vi "Open.vi"(4 "Help URL or File Path":string, 5 "Global Timeout [mSec] (-1)":i32=-1, 6 "Caller VI":refnum<vi>, 7 "Delay [mSec] (0)":u32, 8 "error in (no error)":errorcluster, 9 "Explorer Visible? (F)":bool, 10 "Window Title":string="Action Status", 11 "Bar in":refnum<class "Bar.lvclass">) -> (0 "error out":errorcluster, 3 "Bar out":refnum<class "Bar.lvclass">)   [LabVIEW 2015, in "Simple Progress Bar.lvlib" / "Bar.lvclass"]
doc: "Open the progress bar user interface.\n\n<b>Window Title</b> string will replace the title of the window.\n\n<b>Explorer Visible</b> if enabled will make Explorer button visible. The VI checks if the directory path exists when the event is thrown.\n\n<b>Caller VI</b> reference is used to display progression in the task bar icon (available from Microsoft Windows 7).\n\n<b>Delay</b> in mSec will delay window opening without delaying the process (asynchronous).\n\n<b>Global Timeout</b> duration in mSec will automatically close the window if the process has not finished before."
uses:
  Bar.lvclass
  Bar.lvclass/Bar.ctl
  Simple Progress Bar.lvlib
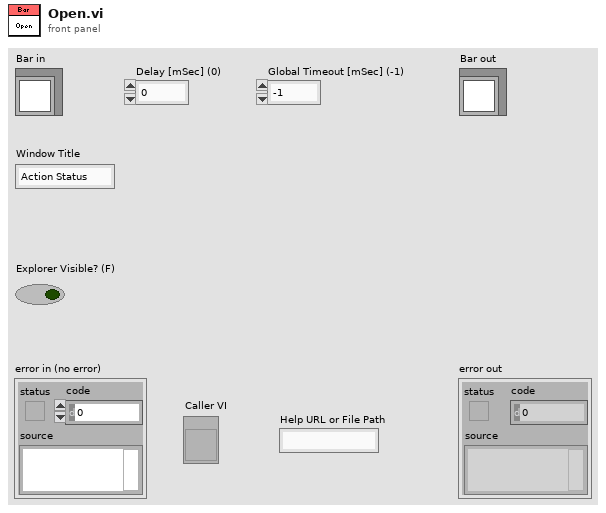
[diagram p1: front panel]
types:
  T1 = enum32{"Invalid", "Standard", "Closed", "Hidden", "Minimized", "Maximized"}
  T2 = typedef "Simple Progress Bar.lvlib/UI Events.ctl" = cluster{"Done":refnum<user-event>, "Cancel":refnum<user-event>, "Explore":refnum<user-event>}
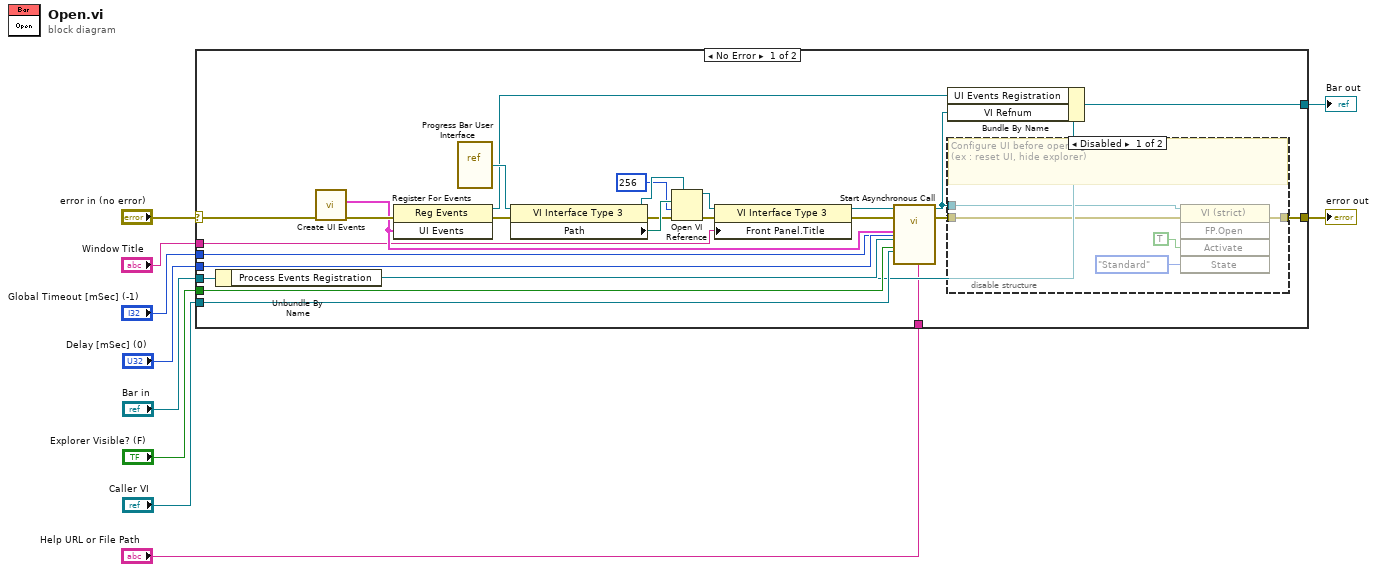
[diagram p0: block diagram]
diagram:
  n1 = case shown="No Error" "error in (no error)" {
    selector: "error in (no error)" -> [w26 w44]
    tunnel: [w30 w44] -> w8
    tunnel: "Explorer Visible? (F)" -> [w25 _]
    tunnel: "Window Title" -> [w20 _]
    tunnel: "Caller VI" -> [w19 _]
    tunnel: "Delay [mSec] (0)" -> [w18 _]
    tunnel: "Bar in" -> [w16 w43]
    tunnel: [w15 w43] -> w3
    tunnel: "Global Timeout [mSec] (-1)" -> [w12 _]
    tunnel: "Help URL or File Path" -> [w11 _]
    frame No Error {
      n2 = Unbundle By Name(w16) -> ("Process Events Registration"=w17:refnum<event-registration>)
      n3 = call "Create UI Events.vi"("error in (no error)"=w26) -> ("error out"=w29:errorcluster, "UI Events"=w27:T2)  [unwired: 9 in]
      n4 = register-events(error in=w29, w27) -> (reference out=w14:refnum<event-registration>, error out=w28:errorcluster)  [unwired: 1 in]
      n5 = vi-ref "Progress Bar User Interface.vi"() -> (w36:refnum<vi>)
      n6 = property class="VI Interface Type 3"(reference=w36, error in=w28) -> (reference out=w33:refnum<vi>, error out=w34:errorcluster, "Path"=w35:path)
      n7 = Open VI Reference(type specifier VI Refnum (for type only)=w33, vi path=w35, options=256, error in (no error)=w34) -> (vi reference=w22:refnum<vi>, error out=w32:errorcluster)  [unwired: 2 in]
      n8 = property class="VI Interface Type 3"(reference=w22, error in=w32, "Front Panel.Title"=w20) -> (reference out=w21:refnum<vi>, error out=w23:errorcluster)
      n9 = call-by-ref "Start Asynchronous Call"(reference=w21, error in=w23, "Help String"=w11, "Global Timeout [mSec] (-1)"=w12, "VI"=w19, "Delay mSec (0)"=w18, "Explorer Visible? (F)"=w25, "Process Events Registration"=w17, "UI Events"=w27) -> (reference out=w13:refnum<vi>, error out=w31:errorcluster)  [unwired: 3 in, 2 out]
      n10 = Bundle By Name(cluster=w16, "UI Events Registration"=w14, "VI Refnum"=w13) -> (w15:refnum<class "Bar.lvclass">)
      n11 = disable-structure shown="Disabled" {
        disable-tunnel: w31 -> [w41 w42]
        disable-tunnel: [w40 w42] -> w30
        disable-tunnel: w13 -> [w39 _]
        frame Disabled {
          # "Configure UI before opening.\n(ex : reset UI, hide explorer)"
          n12 = invoke class="VI (strict)" method="FP.Open"(reference=w39, error in=w41, "Activate"=TRUE ("Activate?"), "State"=T1."Standard") -> (error out=w40:errorcluster)  [unwired: 1 in, 4 out]
        }
        frame Enabled {
        }
      }
    }
    frame Error {
    }
  }
  "error out" <- w8
  "Bar out" <- w3
